vi "SeqEditor_SeqOpen.vi"(8 "error in (no error)":errorcluster, 11 "NLTest in":refnum<class "NLTest.lvclass">) -> (0 "error out":errorcluster, 3 "NLTest out":refnum<class "NLTest.lvclass">)   [LabVIEW 2017, in "NLTest.lvclass"]
uses:
  NLTest.lvclass
  NLTest.lvclass/NLTest.ctl
  VISTEP.ctl
  VISTEP_class_INOUTPUT.ctl
  VISTEP_class_INOUTPUT_TYPE.ctl
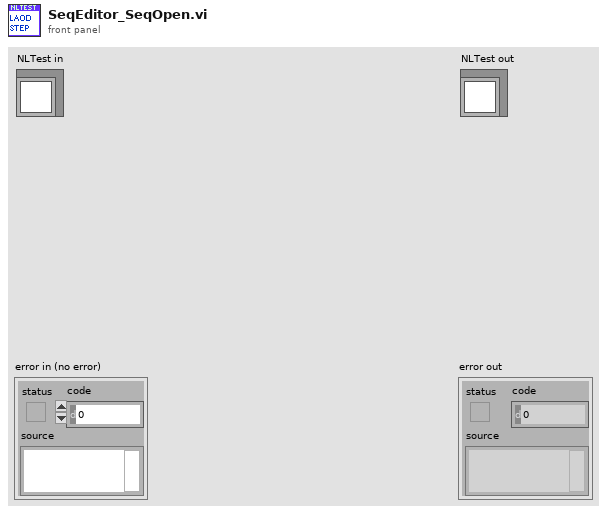
[diagram p1: front panel]
types:
  T1 = typedef "NLTest.lvclass/VISTEP.ctl" = cluster{"My":cluster{"VIpath":T2, "VIname":T2, "Loop":T2, "Skip":T2, "FailStop":T2, "StepClass":T2, "StringTest-Source":T2, "StringTest-Lim":T2, "BoolTest-Source":T2, "BoolTest-Lim":T2, "NumberTest-OP":T2, "NumberTest-Source":T2, "NumberTest-LimA":T2, "NumberTest-LimB":T2}, "INPUT":T2[], "OUTPUT":T2[]}
  T2 = typedef "NLTest.lvclass/VISTEP_class_INOUTPUT.ctl" = cluster{"ITEM":string, "DATA":string, "TYPE":T3, "TYPEDATA":string, "SV":bool, "clusterchain":refnum<vi>[]}
  T3 = typedef "NLTest.lvclass/VISTEP_class_INOUTPUT_TYPE.ctl" = enum16{"Number", "String", "Bool", "Enum", "Path", "VISA", "NA"}
  T4 = typedef "NLTest.lvclass/allseqanddata.ctl" = cluster{"seqname":string, "seqdata":string[]}
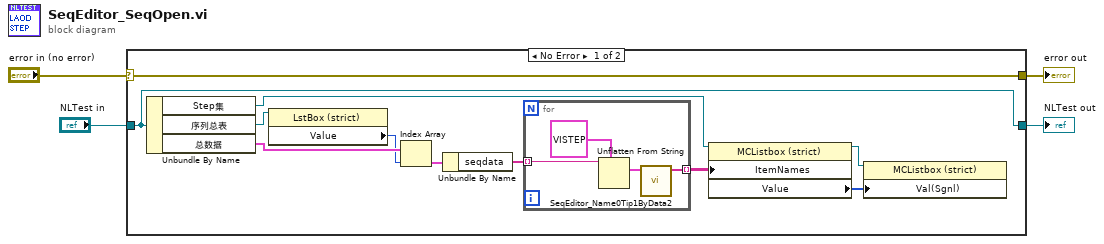
[diagram p0: block diagram]
diagram:
  n1 = case shown="No Error" "error in (no error)" {
    selector: "error in (no error)" -> [w15 w21]
    tunnel: [w15 w21] -> w3
    tunnel: [w14 w20] -> w1
    tunnel: "NLTest in" -> [w14 w20]
    frame No Error {
      n2 = Unbundle By Name(w14) -> ("Step集"=w9:refnum<vi>, "序列总表"=w13:refnum<vi>, "总数据"=w12:T4[])
      n3 = property class="LstBox (strict)"(reference=w13) -> ("Value"=w11:i32)  [unwired: 1 in, 2 out]
      n4 = Index Array(array=w12, index=w11) -> (element=w10:T4)
      n5 = Unbundle By Name(w10) -> ("seqdata"=w8:string[])
      n6 = for {
        tunnel: w8 -> [w18] mode=indexing
        tunnel: [w16] -> w7 mode=indexing
        n7 = Unflatten From String(type=T1 {"My"={"VIpath"={"ITEM"="VI路径", "DATA"="", "TYPE"=enum."Path", "TYPEDATA"="", "SV"=FALSE, "clusterchain"=[]}, "VIname"={"ITEM"="步骤名称", "DATA"="", "TYPE"=enum."String", "TYPEDATA"="", "SV"=FALSE, "clusterchain"=[]}, "Loop"={"ITEM"="重测次数", "DATA"="1", "TYPE"=enum."Number", "TYPEDATA"="", "SV"=FALSE, "clusterchain"=[]}, "Skip"={"ITEM"="跳过步骤", "DATA"="FALSE", "TYPE"=enum."Bool", "TYPEDATA"="", "SV"=FALSE, "clusterchain"=[]}, "FailStop"={"ITEM"="失败停止", "DATA"="FALSE", "TYPE"=enum."Bool", "TYPEDATA"="", "SV"=FALSE, "clusterchain"=[]}, "StepClass"={"ITEM"="步骤类型", "DATA"="NotaTEST", "TYPE"=enum."Enum", "TYPEDATA"="", "SV"=FALSE, "clusterchain"=[]}, "StringTest-Source"={"ITEM"="字符串测试值", "DATA"="", "TYPE"=enum."String", "TYPEDATA"="", "SV"=FALSE, "clusterchain"=[]}, "StringTest-Lim"={"ITEM"="字符串测试门限", "DATA"="", "TYPE"=enum."String", "TYPEDATA"="", "SV"=FALSE, "clusterchain"=[]}, "BoolTest-Source"={"ITEM"="布尔测试值", "DATA"="", "TYPE"=enum."Bool", "TYPEDATA"="", "SV"=FALSE, "clusterchain"=[]}, "BoolTest-Lim"={"ITEM"="布尔测试门限", "DATA"="", "TYPE"=enum."Bool", "TYPEDATA"="", "SV"=FALSE, "clusterchain"=[]}, "NumberTest-OP"={"ITEM"="数值测试OP", "DATA"="", "TYPE"=enum."Enum", "TYPEDATA"="", "SV"=FALSE, "clusterchain"=[]}, "NumberTest-Source"={"ITEM"="数值测试值", "DATA"="", "TYPE"=enum."Number", "TYPEDATA"="", "SV"=FALSE, "clusterchain"=[]}, "NumberTest-LimA"={"ITEM"="数值测试门限A", "DATA"="", "TYPE"=enum."Number", "TYPEDATA"="", "SV"=FALSE, "clusterchain"=[]}, "NumberTest-LimB"={"ITEM"="数值测试门限B", "DATA"="", "TYPE"=enum."Number", "TYPEDATA"="", "SV"=FALSE, "clusterchain"=[]}}, "INPUT"=[], "OUTPUT"=[]} ("步骤结构"), binary string=w18) -> (value=w17:T1)  [unwired: 3 in, 2 out]
        n8 = call "SeqEditor_Name0Tip1ByData2.vi"("output cluster"=w17) -> ("Array"=w16:string[])  [unwired: 10 in]
      }
      n9 = property class="MCListbox (strict)"(reference=w9, "ItemNames"=w7) -> (reference out=w6:refnum<vi>, "Value"=w5:i32[])  [unwired: 1 in, 1 out]
      n10 = property class="MCListbox (strict)"(reference=w6, "Val(Sgnl)"=w5) -> ()  [unwired: 1 in, 2 out]
    }
    frame Error {
    }
  }
  "error out" <- w3
  "NLTest out" <- w1
